vi "Create User Event - Stop.vi"(8 "error in (no error)":errorcluster) -> (0 "error out":errorcluster, 3 "User events":T1)   [LabVIEW 2020, in "oled User Event - Stop.lvlib"]
doc: "Create a boolean user event that will be used to stop the event loop from the message handling loop."
uses:
  oled User Event - Stop.lvlib
  controls/HL Acq Data.ctl
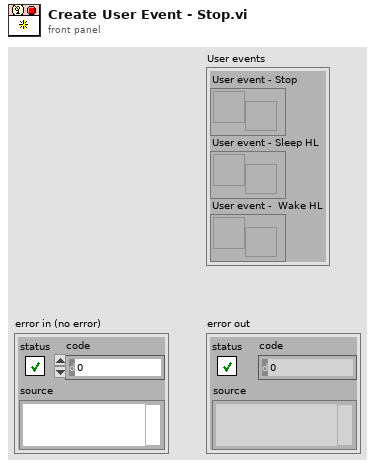
[diagram p1: front panel]
types:
  T1 = cluster{"User event - Stop":refnum<user-event>, "User event - Sleep HL":refnum<user-event>, "User event -  Wake HL":refnum<user-event>}
  T2 = typedef "HL Acq Data.ctl" = cluster{"dV":dbl, "Vmax":dbl, "Vo":dbl}
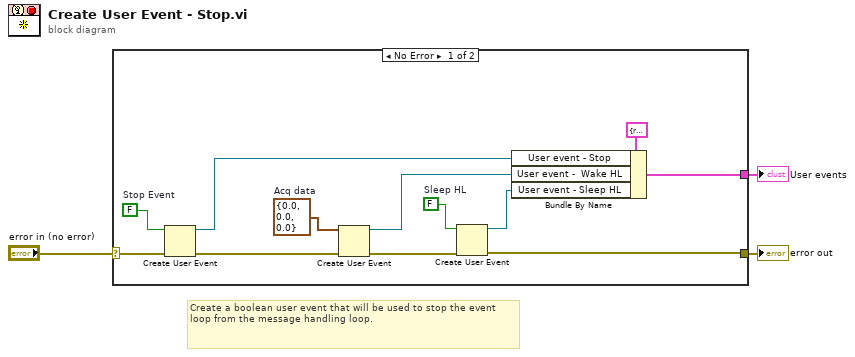
[diagram p0: block diagram]
diagram:
  # "Create a boolean user event that will be used to stop the event loop from the message handling loop."
  n1 = case shown="No Error" "error in (no error)" {
    selector: "error in (no error)" -> [w14 w16]
    tunnel: [w11 w16] -> w3
    tunnel: [w7 _] -> w1
    frame No Error {
      w4 = T2 {"dV"=0.0, "Vmax"=0.0, "Vo"=0.0}  # Acq data
      w8 = FALSE  # Sleep HL
      w15 = FALSE  # Stop Event
      n2 = Create User Event(user event datatype=w15, error in=w14) -> (user event=w6:refnum<user-event>, error out=w13:errorcluster)
      n3 = Create User Event(user event datatype=w4, error in=w13) -> (user event=w9:refnum<user-event>, error out=w12:errorcluster)
      n4 = Create User Event(user event datatype=w8, error in=w12) -> (user event=w10:refnum<user-event>, error out=w11:errorcluster)
      n5 = Bundle By Name(cluster=T1 {"User event - Stop"=refnum, "User event - Sleep HL"=refnum, "User event -  Wake HL"=refnum}, "User event - Stop"=w6, "User event -  Wake HL"=w9, "User event - Sleep HL"=w10) -> (w7:T1)
    }
    frame Error {
    }
  }
  "error out" <- w3
  "User events" <- w1
